vi "Tx.vi"() -> ()   [LabVIEW 2015]
uses:
  <instrlib>/niUSRP/niUSRP Write Tx Data (CDB).vi
panel:
  in  "dimension size":i32
  out "error out":errorcluster
  out "coerced gain":dbl format="%#_6f"
  out "coerced carrier frequency":dbl=100000.0 format="%#_6p"
  out "coerced IQ rate":dbl=100000.0 format="%#_6p"
  in  "active antenna":string
  in  "IQ rate":dbl=100000.0 format="%#_6p"
  in  "gain":dbl format="%#_6f"
  in  "carrier frequency":dbl=100000.0 format="%#_6p"
  in  "device names":refnum<k15>
  in  "stop":bool
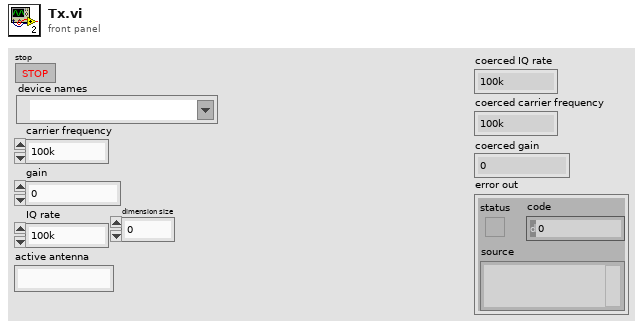
[diagram p1: front panel]
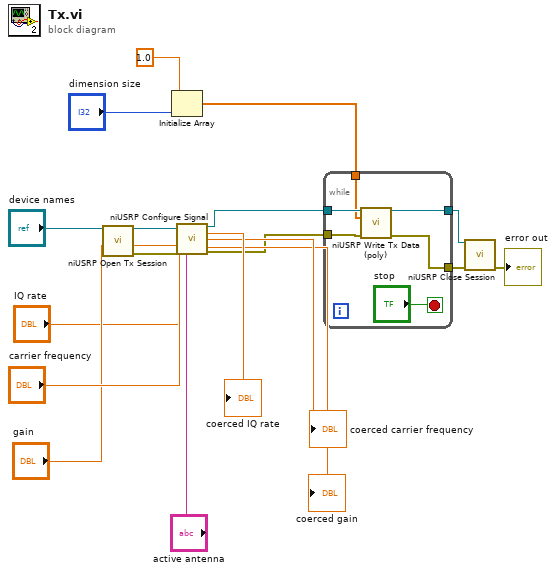
[diagram p0: block diagram]
diagram:
  n1 = call <instrlib>:"niUSRP Open Tx Session.vi"("device names"="device names") -> ("session handle out"=w10:refnum<k15>, "error out"=w7:errorcluster)  [unwired: 13 in]
  n2 = Initialize Array(1.0 ("element"), "dimension size") -> (w1:dbl[])
  n3 = call <instrlib>:"niUSRP Configure Signal.vi"("session handle"=w10, "IQ rate"="IQ rate", "carrier frequency"="carrier frequency", "gain"="gain", "error in (no error)"=w7, "active antenna"="active antenna") -> ("session handle out"=w9:refnum<k15>, "coerced IQ rate"=→"coerced IQ rate":dbl, "coerced carrier frequency"=→"coerced carrier frequency":dbl, "coerced gain"=→"coerced gain":dbl, "error out"=w6:errorcluster)  [unwired: 5 in]
  n4 = while {
    tunnel: w9 -> [w23]
    tunnel: [w22] -> w8
    tunnel: w6 -> [w21]
    tunnel: [w20] -> w5
    tunnel: w1 -> [w19]
    stop <- "stop" stop-if-true
    n5 = call-poly <instrlib>:"niUSRP Write Tx Data (poly).vi"("session handle"=w23, "data"=w19, "error in (no error)"=w21) -> ("session handle out"=w22:refnum<k15>, "error out"=w20:errorcluster)  [unwired: 11 in]
  }
  n6 = call <instrlib>:"niUSRP Close Session.vi"("session handle"=w8, "error in (no error)"=w5) -> ("error out"=→"error out":errorcluster)  [unwired: 13 in]
